vi "sort channels.vi"(8 "error in (no error)":errorcluster, 11 "channels in":refnum<class "TBM channel.lvclass">[](array[class])) -> (0 "error out":errorcluster, 3 "channels out":refnum<class "TBM channel.lvclass">[](array[class]))   [LabVIEW 2014, in "Shared Memory configuration.lvclass"]
uses:
  module/configuration/Shared Memory configuration.lvclass
  <vilib>/NI/Tag Bus Module Framework/channel/TBM channel.lvclass
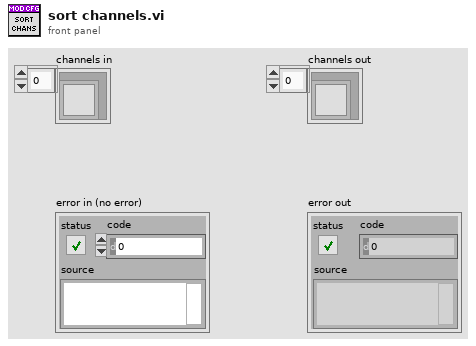
[diagram p1: front panel]
types:
  T1 = typedef "tag bus.lvlib/tag descriptor.lvclass/Data Type.ctl" = enum16{"Double", "Single", "I64", "I32", "I16", "I8", "U64", "U32", "U16", "U8", "Boolean", "String", "Array of Double", "Array of Single", "Array of I64", "Array of I32", "Array of I16", "Array of I8", "Array of U64", "Array of U32", "Array of U16", "Array of U8", "Array of Boolean", "Array of String"}
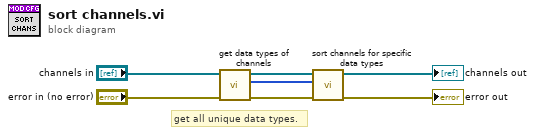
[diagram p0: block diagram]
diagram:
  # "get all unique data types."
  n1 = call "get data types of channels.vi"("error in (no error)"="error in (no error)", "channels in"="channels in") -> ("error out"=w5:errorcluster, "data types"=w1:T1[], "channels out"=w2:refnum<class "TBM channel.lvclass">[])  [unwired: 7 in]
  n2 = call "sort channels for specific data types.vi"("error in (no error)"=w5, "data types"=w1, "channels in"=w2) -> ("error out"=→"error out":errorcluster, "channels out"=→"channels out":refnum<class "TBM channel.lvclass">[])  [unwired: 7 in]
